vi "libssh2_userauth_list.vi"(8 "error in (no error)":errorcluster, 10 "username":string, 11 "session":T1) -> (0 "error out":errorcluster, 2 "supported authentication schemes":string)   [LabVIEW 2017, in "libssh2.lvlib"]
doc: "Get a list of authentication methods that are available for a session.\n\nSends a SSH_USERAUTH_NONE request to the remote host. Unless the remote is configured to accept \"none\" as a viable authentication scheme, it will return SSH_USERAUTH_FAILURE along with a listing of what authentication schemes it does support. In the unlikely event that none-authentication succeeds, this method returns an empty string. This can be distinguished from a failing case by examining <B>libssh2_userauth_authenticated</B>."
uses:
  libssh2.lvlib
  Session Refnum.ctl
  Not A Session.vi
  <vilib>/Utility/error.llb/Error Cluster From Error Code.vi
  Global Settings.vi
  Read Session Refnum.vi
  <vilib>/Utility/semaphor.llb/Acquire Semaphore.vi
  <vilib>/Utility/semaphor.llb/Release Semaphore.vi
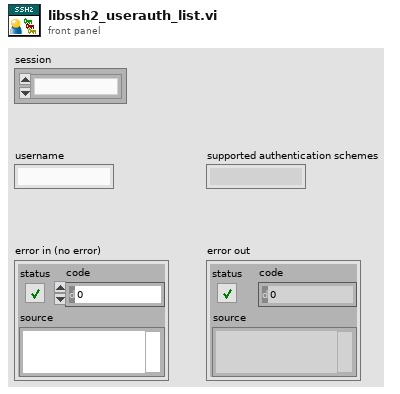
[diagram p1: front panel]
types:
  T1 = typedef "libssh2.lvlib/Session Refnum.ctl" = refnum<k1>
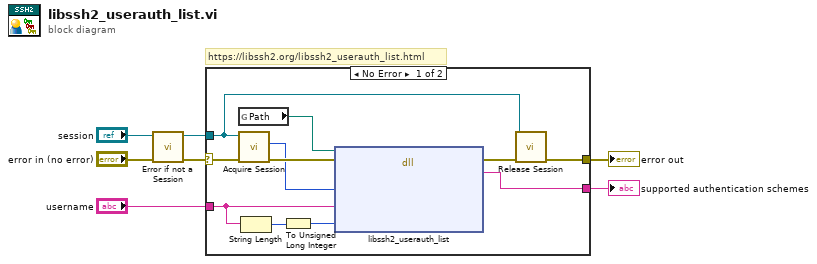
[diagram p0: block diagram]
diagram:
  # "https://libssh2.org/libssh2_userauth_list.html"
  n1 = call "Error if not a Session.vi"("error in (no error)"="error in (no error)", "session"="session") -> ("error out"=w3:errorcluster, "session out"=w1:T1)  [unwired: 8 in]
  n2 = case shown="No Error" w3 {
    selector: w3 -> [w15 w19]
    tunnel: "username" -> [w18 _]
    tunnel: [w17 _] -> w6
    tunnel: [w9 w19] -> w5
    tunnel: w1 -> [w8 _]
    frame No Error {
      n3 = global read "Global Settings.vi" "Path"() -> (w10:path)
      n4 = call "Acquire Session.vi"("error in (no error)"=w15, "session"=w8) -> ("error out"=w12:errorcluster, "LIBSSH2_SESSION*"=w11:u64)  [unwired: 7 in, 1 out]
      n5 = String Length(string=w18) -> (length=w13:i32)
      n6 = To Unsigned Long Integer(number=w13) -> (unsigned 32bit integer=w14:u32)
      n7 = dll-call lib="?" fn="libssh2_userauth_list"(path in=w10, error in=w12, "session"=w11, "username"=w18, "username_len"=w14) -> (error out=w16:errorcluster, "return value"=w17:string)  [unwired: 4 in, 1 out]
      n8 = call "Release Session.vi"("error in (no error)"=w16, "session"=w8) -> ("error out"=w9:errorcluster)  [unwired: 9 in]
    }
    frame Error {
    }
  }
  "supported authentication schemes" <- w6
  "error out" <- w5
